vi "PicoScope3000aGetTimebase2.vi"(4 "Number of Samples":u32, 6 "Memory Segment":u32, 7 "Acquisition Settings":T1={"preTriggerSamples"=0, "postTriggerSamples"=5000000, "timebase"=5} {"postTriggerSamples" format="%_6p"; "preTriggerSamples" format="%_6p"}, 8 "error in (no error)":errorcluster, 11 "handle in":i16) -> (0 "error out":errorcluster, 3 "handle out":i16, 5 "Properties Panel":T2 {"Max Total Capture Time Available (sec)" format="%.3p"; "Sample Frequency" format="%.3p"; "Sample Rate" format="%.3p"; "Max Samples Available" format="%.3p"; "Total Capture Time (sec)" format="%.3p"})   [LabVIEW 2010]
uses:
  ps3000a.dll
  shared/Acquisition Settings.ctl
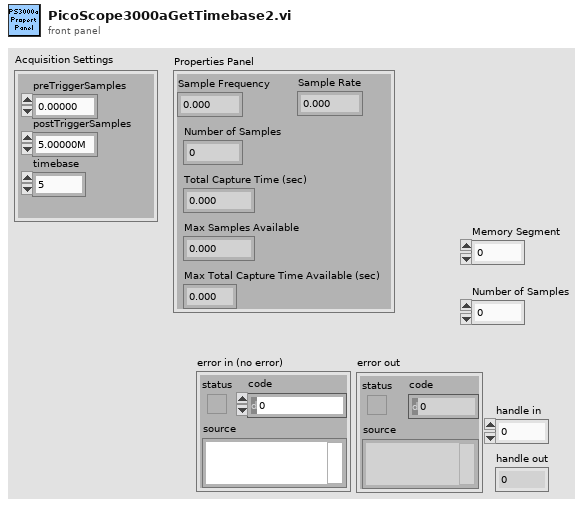
[diagram p1: front panel]
types:
  T1 = typedef "Acquisition Settings.ctl" = cluster{"preTriggerSamples":u64, "postTriggerSamples":u64, "timebase":u32}
  T2 = cluster{"Sample Frequency":sgl, "Sample Rate":sgl, "Max Samples Available":i32, "Number of Samples":u32, "Total Capture Time (sec) ":sgl, "Max Total Capture Time Available (sec)":sgl}
  T3 = cluster{sgl, sgl, "maxSamples":i32, "Number of Samples":u32, sgl, sgl}
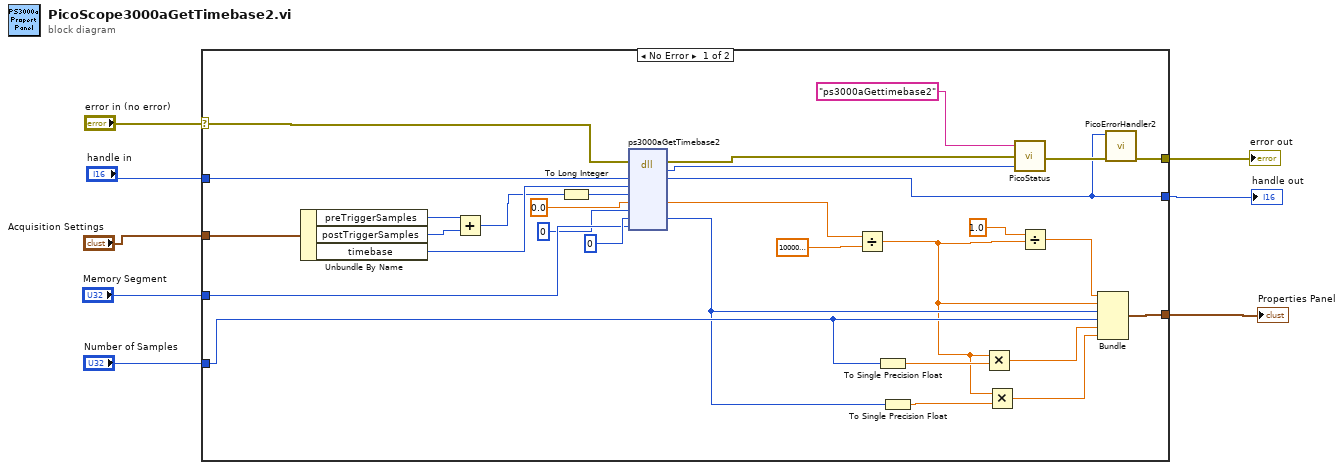
[diagram p0: block diagram]
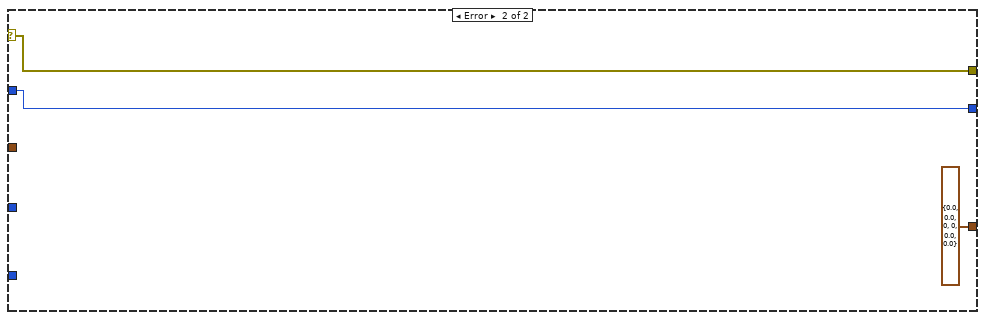
[diagram p2: hidden frame]
diagram:
  n1 = case shown="No Error" "error in (no error)" {
    selector: "error in (no error)" -> [w12 w41]
    tunnel: [w11 w41] -> w8
    tunnel: [w9 w40] -> w7
    tunnel: "Memory Segment" -> [w29 _]
    tunnel: "Number of Samples" -> [w24 _]
    tunnel: "handle in" -> [w28 w40]
    tunnel: "Acquisition Settings" -> [w27 _]
    tunnel: [w20 T3 {0.0, 0.0, "maxSamples"=0, "Number of Samples"=0, 0.0, 0.0}] -> w2
    frame No Error {
      n2 = Unbundle By Name(w27) -> ("preTriggerSamples"=w33:u64, "postTriggerSamples"=w34:u64, "timebase"=w35:u32)
      n3 = Add(x=w33, y=w34) -> (x+y=w14:u64)
      n4 = To Long Integer(number=w14) -> (32bit integer=w15:i32)
      n5 = dll-call lib="ps3000a.dll" fn="ps3000aGetTimebase2"(error in=w12, "handle"=w28, "timebase"=w35, "noSamples"=w15, "timeIntervalNanoseconds"=sgl 0.0, "oversample"=i16 0, "maxSamples"=0, "segmentIndex"=w29) -> (error out=w36:errorcluster, "PICO_STATUS"=w30:u32, "handle"=w9:i16, "timeIntervalNanoseconds"=w37:sgl, "maxSamples"=w22:i32)  [unwired: 6 in, 1 out]
      n6 = Divide(x=w37, y=sgl 1000000000.0) -> (x/y=w19:sgl)
      n7 = To Single Precision Float(number=w24) -> (single precision float=w26:sgl)
      n8 = To Single Precision Float(number=w22) -> (single precision float=w23:sgl)
      n9 = Multiply(x=w19, y=w26) -> (x*y=w25:sgl)
      n10 = Multiply(x=w19, y=w23) -> (x*y=w21:sgl)
      n11 = call "PicoStatus.vi"("PICO STATUS"=w30, "error in"=w36, "source"="ps3000aGettimebase2") -> ("error out"=w10:errorcluster)
      n12 = Divide(x=sgl 1.0, y=w19) -> (x/y=w17:sgl)
      n13 = Bundle(w17, w19, "maxSamples"=w22, "Number of Samples"=w24, w25, w21) -> (w20:T3)  [unwired: 1 in]
      n14 = call "PicoErrorHandler2.vi"("error in (no error)"=w10, "handle In"=w9) -> ("error out"=w11:errorcluster)  [unwired: 9 in]
    }
    frame Error {
    }
  }
  "error out" <- w8
  "handle out" <- w7
  "Properties Panel" <- w2
